vi "IRdata.vi"(2 "error in (no error)":errorcluster) -> (0 "error out":errorcluster)   [LabVIEW 2019]
uses:
  <vilib>/myRIO/Instrument Drivers/Onboard IO/AI/typedefs/AI Reference.ctl
  <vilib>/myRIO/Common/Instrument Driver Framework/Utilities/typedefs/myRIO Generic Hardware Reference.ctl
  <vilib>/myRIO/Common/Instrument Driver Framework/Utilities/typedefs/Hardware Version Enum.ctl
  <vilib>/myRIO/Common/Instrument Driver Framework/Utilities/typedefs/myRIO v1.0 Reference.ctl
  <vilib>/myRIO/Common/Instrument Driver Framework/Utilities/typedefs/Generic FPGA Reference.ctl
  <vilib>/myRIO/Common/Instrument Driver Framework/myRIO v1.0/AI/typedefs/AI Channels List.ctl
  <vilib>/myRIO/Common/Instrument Driver Framework/myRIO v1.0/AI/typedefs/AI Channels Enum.ctl
  <vilib>/myRIO/Common/Instrument Driver Framework/Utilities/typedefs/Analog Scaling Constants List.ctl
  <vilib>/myRIO/Common/Instrument Driver Framework/Utilities/typedefs/Analog Scaling Constants.ctl
  <vilib>/userDefined/High Color/nirio_resource_hc.ctl
  <vilib>/myRIO/Common/Instrument Driver Framework/Utilities/vis/Is FPGA Ref Available.vi
  <vilib>/myRIO/Common/Instrument Driver Framework/myRIO v1.0/AI/vis/myRIO v1.1 Open AI.vi
  <vilib>/myRIO/Instrument Drivers/Onboard IO/AI/vis/Read.vi
  <vilib>/myRIO/Common/Instrument Driver Framework/Utilities/vis/Validate Channels.vi
  <vilib>/myRIO/Common/Instrument Driver Framework/myRIO v1.0/AI/vis/myRIO v1.0 Reserve AI.vi
  <vilib>/myRIO/Common/Instrument Driver Framework/myRIO v1.0/AI/vis/myRIO v1.0 Build MUX Configuration AI.vi
  <vilib>/myRIO/Common/Instrument Driver Framework/myRIO v1.0/Resource Manager/vis/myRIO v1.0 Reserve Channel List.vi
  <vilib>/myRIO/Common/Instrument Driver Framework/myRIO v1.0/Resource Manager/vis/myRIO v1.0 Reserve Channel.vi
  <vilib>/myRIO/Common/Instrument Driver Framework/myRIO v1.0/Resource Manager/vis/myRIO v1.0 Unreserve Channel.vi
  <vilib>/myRIO/Common/Instrument Driver Framework/myRIO v1.0/Resource Manager/vis/myRIO v1.0 Build Mutex Name.vi
  <vilib>/Utility/VariantDataType/GetNumericInfo.vi
  <vilib>/Utility/error.llb/Error Cluster From Error Code.vi
  <vilib>/myRIO/Common/Instrument Driver Framework/myRIO v1.0/myRIO v1.1 Open.vi
  <vilib>/myRIO/Common/Instrument Driver Framework/myRIO v1.0/AI/vis/myRIO v1.0 Get Scaling Constants AI.vi
  <vilib>/myRIO/Common/Instrument Driver Framework/Utilities/vis/IO Manager.vi
  <vilib>/myRIO/Common/Instrument Driver Framework/Utilities/vis/Configuration Manager.vi
  <vilib>/myRIO/Common/Instrument Driver Framework/myRIO v1.0/myRIO v1.0 Close.vi
  <vilib>/myRIO/Common/Instrument Driver Framework/myRIO v1.0/AI/vis/myRIO v1.0 Read AI.vi
  <vilib>/myRIO/Express VI/Onboard IO/AI/AI Express VI.xnode
  <vilib>/myRIO/Instrument Drivers/Onboard IO/AI/vis/myRIO AI Open.xnode
  <vilib>/myRIO/Instrument Drivers/Onboard IO/AI/AI.lvlib
  <vilib>/ptbypt/NI_PtbyPt.lvlib
panel:
  in  "stop":bool
  out "紅外線數值 2":T1
  in  "Boolean":bool
  out "紅外線數值":T1
  in  "右前參數":cluster{"m":dbl, "b":dbl, "k":dbl}={"m"=0.0361037, "b"=0.0354848, "k"=4.28571}
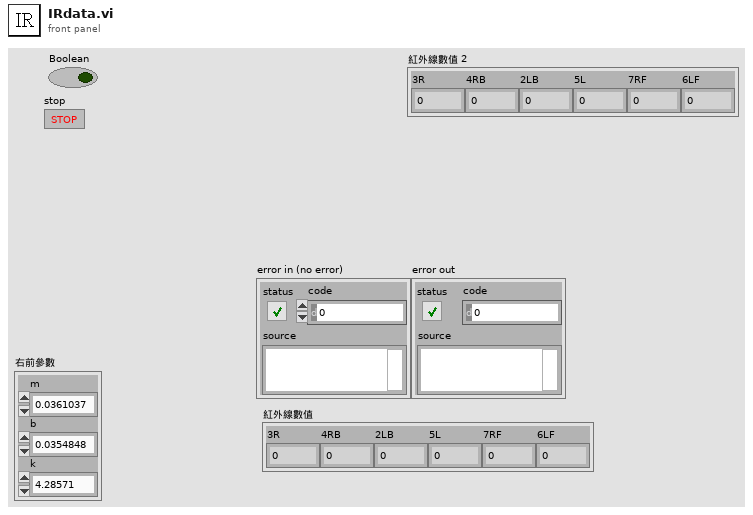
[diagram p1: front panel]
types:
  T1 = cluster{"7RF":dbl, "3R":dbl, "4RB":dbl, "5L":dbl, "6LF":dbl, "2LB":dbl}
  T2 = typedef "AI.lvlib/AI Reference.ctl" = cluster{"myRIO Reference":T3, "AI Channels List":T7, "AI Scaling Constants List":T9}
  T3 = typedef "myRIO Generic Hardware Reference.ctl" = cluster{"myRIO Model":T4, "myRIO Hardware Reference":T5}
  T4 = typedef "Hardware Version Enum.ctl" = enum16{"Unknown", "myRIO-1900", "myRIO-1950", "roboRIO", "NI ELVIS RIO CM", "ELVIS III"}
  T5 = typedef "myRIO v1.0 Reference.ctl" = cluster{"Generic FPGA Reference":T6, "Allow multiple opens":bool}
  T6 = typedef "Generic FPGA Reference.ctl" = refnum<k20>
  T7 = typedef "AI Channels List.ctl" = T8[]
  T8 = typedef "AI Channels Enum.ctl" = enum16{"Not Connected", "AudioIn/Left", "AudioIn/Right", "C/AI0", "C/AI1", "A/AI0", "A/AI1", "A/AI2", "A/AI3", "A/AI4", "A/AI5", "A/AI6", "A/AI7", "B/AI0", "B/AI1", "B/AI2", "B/AI3", "B/AI4", "B/AI5", "B/AI6", "B/AI7", "AI/AI0", "AI/AI1", "AI/AI2", "AI/AI3", "A/AI0 (DIFF)", "A/AI1 (DIFF)", "A/AI2 (DIFF)", "A/AI3 (DIFF)", "B/AI0 (DIFF)", "B/AI1 (DIFF)", "B/AI2 (DIFF)", "B/AI3 (DIFF)"}
  T9 = typedef "Analog Scaling Constants List.ctl" = T10[]
  T10 = typedef "Analog Scaling Constants.ctl" = cluster{"LSB Weight (Volts)":dbl, "Offset (Volts)":dbl, "Signed?":bool}
  T11 = typedef "nirio_resource_hc.ctl" = tag
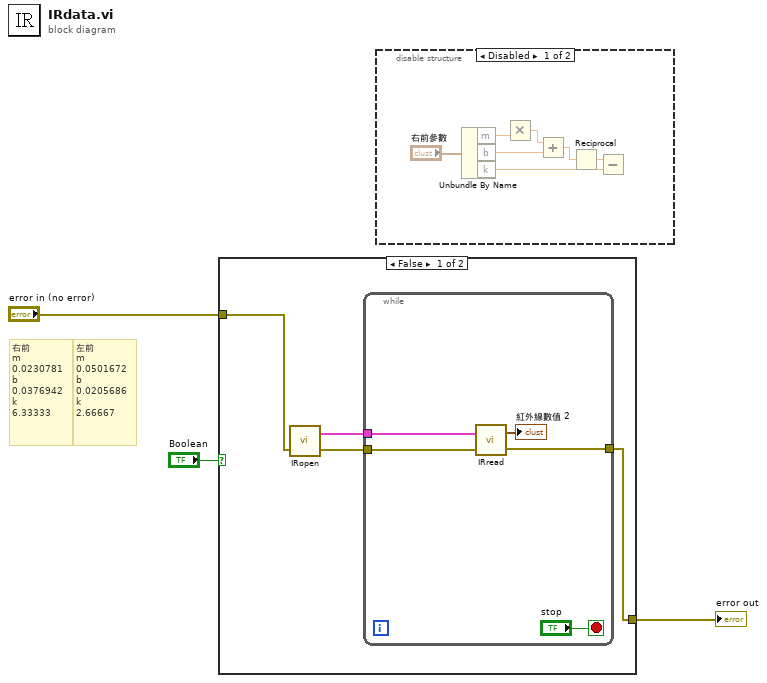
[diagram p0: block diagram]
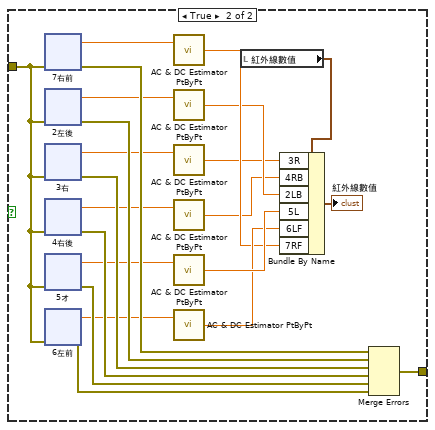
[diagram p2: hidden frame]
diagram:
  # "右前\nm\n0.0230781\nb\n0.0376942\nk\n6.33333"
  # "左前\nm\n0.0501672\nb\n0.0205686\nk\n2.66667"
  n1 = case shown="False" "Boolean" {
    tunnel: "error in (no error)" -> [w7 w34]
    tunnel: [w4 w27] -> w2
    frame False {
      n2 = call "IRopen.vi"("error in (no error)"=w7) -> ("error out"=w5:errorcluster, "AI Ref Out"=w6:T2)  [unwired: 1 in]
      n3 = while {
        tunnel: w6 -> [w12]
        tunnel: w5 -> [w11]
        tunnel: [w9] -> w4
        stop <- "stop" stop-if-true
        n4 = call "IRread.vi"("error in (no error)"=w11, "AI Ref In"=w12) -> ("error out"=w9:errorcluster, "紅外線數值"=→"紅外線數值 2":T1)
      }
    }
    frame True {
      n5 = xnode "7右前"("error in (no error)"=w34) -> ("error out"=w28:errorcluster, "A/AI3 (Pin 9)"=w24:dbl)
      n6 = xnode "2左後"("error in (no error)"=w34) -> ("error out"=w29:errorcluster, "A/AI2 (Pin 7)"=w18:dbl)
      n7 = xnode "3右"("error in (no error)"=w34) -> ("error out"=w30:errorcluster, "A/AI1 (Pin 5)"=w16:dbl)
      n8 = xnode "4右後"("error in (no error)"=w34) -> ("error out"=w31:errorcluster, "A/AI0 (Pin 3)"=w14:dbl)
      n9 = xnode "5オ"("error in (no error)"=w34) -> ("error out"=w32:errorcluster, "B/AI3 (Pin 9)"=w22:dbl)
      n10 = xnode "6左前"("error in (no error)"=w34) -> ("error out"=w33:errorcluster, "B/AI2 (Pin 7)"=w23:dbl)
      n11 = call <vilib>:"AC & DC Estimator PtByPt.vi"("signal"=w24) -> ("DC estimate (V)"=w19:dbl)  [unwired: 2 in, 2 out]
      n12 = call <vilib>:"AC & DC Estimator PtByPt.vi"("signal"=w18) -> ("DC estimate (V)"=w17:dbl)  [unwired: 2 in, 2 out]
      n13 = call <vilib>:"AC & DC Estimator PtByPt.vi"("signal"=w16) -> ("DC estimate (V)"=w15:dbl)  [unwired: 2 in, 2 out]
      n14 = call <vilib>:"AC & DC Estimator PtByPt.vi"("signal"=w14) -> ("DC estimate (V)"=w13:dbl)  [unwired: 2 in, 2 out]
      n15 = call <vilib>:"AC & DC Estimator PtByPt.vi"("signal"=w22) -> ("DC estimate (V)"=w21:dbl)  [unwired: 2 in, 2 out]
      n16 = call <vilib>:"AC & DC Estimator PtByPt.vi"("signal"=w23) -> ("DC estimate (V)"=w20:dbl)  [unwired: 2 in, 2 out]
      n17 = local read "紅外線數值"() -> (w25:T1)
      n18 = Bundle By Name(cluster=w25, "3R"=w15, "4RB"=w13, "2LB"=w17, "5L"=w21, "6LF"=w20, "7RF"=w19) -> (→"紅外線數值":T1)
      n19 = Merge Errors(w28, w29, w30, w31, w32, w33) -> (w27:errorcluster)
    }
  }
  "error out" <- w2
  n20 = disable-structure shown="Disabled" {
    frame Disabled {
      n21 = Unbundle By Name("右前參數") -> ("m"=w260:dbl, "b"=w261:dbl, "k"=w262:dbl)
      n22 = Multiply(y=w260) -> (x*y=w257:dbl)  [unwired: 1 in]
      n23 = Add(x=w257, y=w261) -> (x+y=w259:dbl)
      n24 = Reciprocal(x=w259) -> (1/x=w258:dbl)
      n25 = Subtract(x=w258, y=w262) -> ()  [unwired: 1 out]
    }
    frame Enabled {
    }
  }
